vi "_Pull Controls Value to DPs(VI).vi"(6 "sync DPs?(T)":bool=TRUE, 7 "VIRef(Caller VI)":refnum<vi>, 8 "error in (no error)":errorcluster, 9 "force update(F)":bool, 11 "SILAPI In":refnum<k1>) -> (0 "error out":errorcluster, 1 "Binded DPs":string[](array[string]), 3 "SILAPI Out":refnum<k1>)   [LabVIEW 2017, in "TagDB RefManager.lvlib"]
uses:
  TagDB RefManager.lvlib
  230c0da9-b6e4-44e0-8cb2-fe6bdec026ba.vi
  e135edd7-4a87-4b9d-b0c7-3b3f0cd11366.vi
  be640558-f0fc-44bb-96cd-108508b5fbdb.vi
  083faeab-0307-4387-9797-c882d96e285b.vi
  a032c900-6a26-4ad4-8296-bdd15205f1fc.vi
  024ec822-42c1-4cee-abf5-dbe2fbe4f70a.vi
  <userlib>/_NEVSTOP/TagDB/_Support/DataAccess/_NameCacher.vi
  <userlib>/_NEVSTOP/TagDB/_Support/Error/_[error50002]Invalid DataType.vi
  <userlib>/_NEVSTOP/TagDB/_Support/Error/_[error50000]Invalid DB REF.vi
  <userlib>/_NEVSTOP/TagDB/_Support/DataAccess/TagDB Ref to DVR.vi
  <userlib>/_NEVSTOP/TagDB/_Support/URL/TRIM-BOTH-SPACE.vi
  <userlib>/_NEVSTOP/TagDB/_Support/DataAccess/data-Write.vi
  <userlib>/_NEVSTOP/TagDB/_Support/DataAccess/_datatypeChecker.vi
  <userlib>/_NEVSTOP/TagDB/_Support/Error/_Build Error Cluster.vi
  <vilib>/Utility/Data Type/Get Type Information.vi
  <userlib>/_NEVSTOP/TagDB/TagDB.lvlib
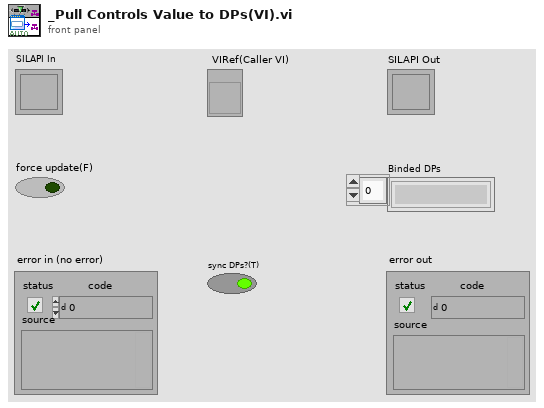
[diagram p1: front panel]
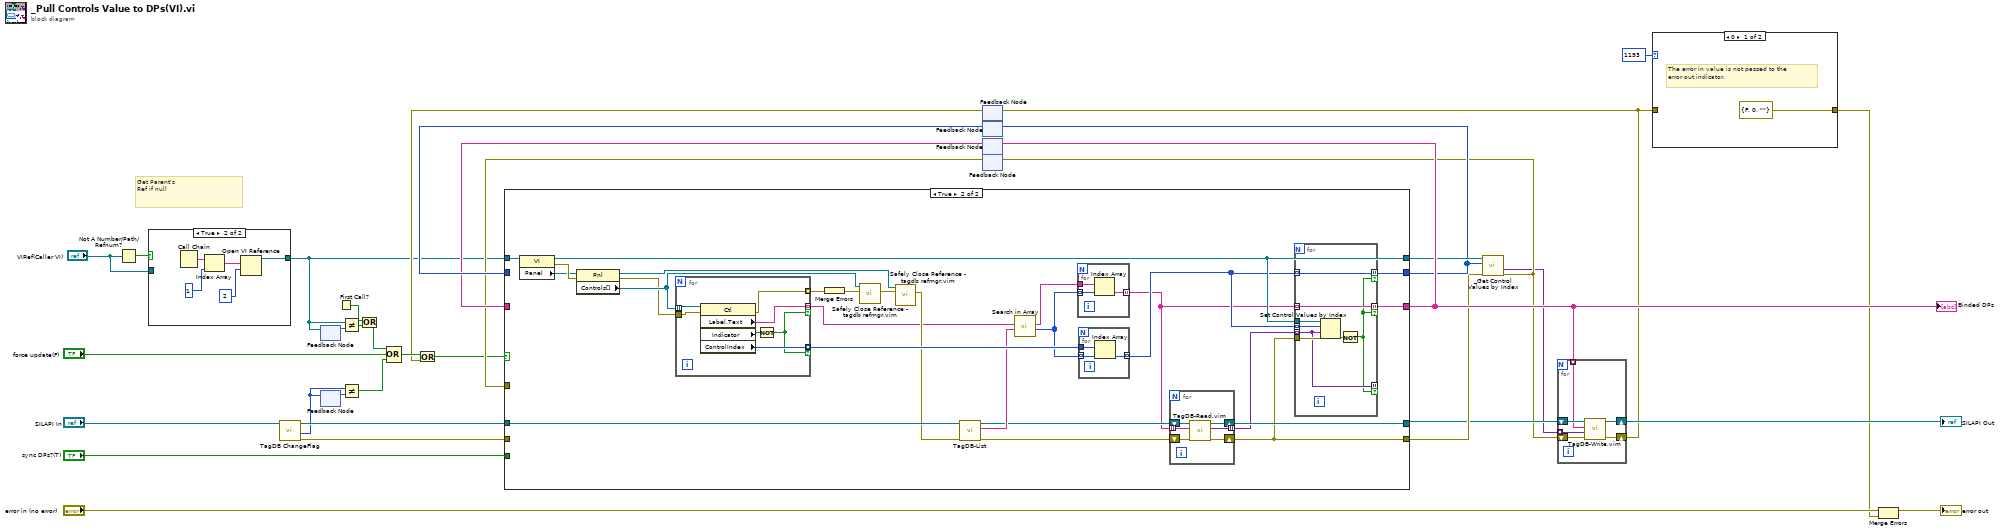
[diagram p0: block diagram]
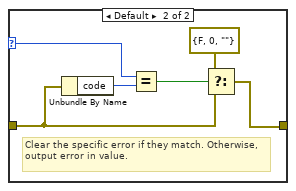
[diagram p3: hidden frame]
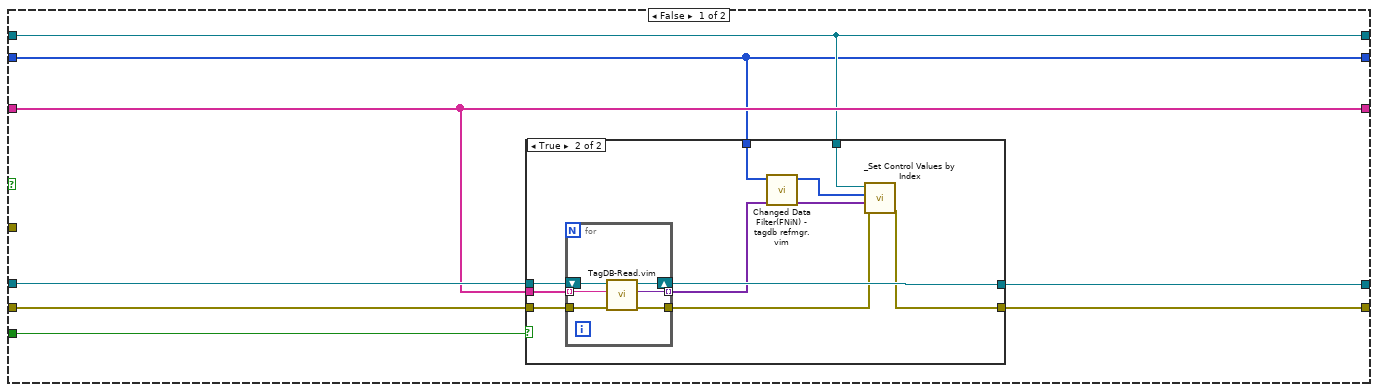
[diagram p4: hidden frame]
diagram:
  # "Get Parent's\nRef if null"
  n1 = Not A Number/Path/Refnum?(number/path/refnum="VIRef(Caller VI)") -> (NaN/Path/Refnum?=w13:bool)
  n2 = case shown="True" w13 {
    tunnel: [w35 w36] -> w8
    tunnel: "VIRef(Caller VI)" -> [w35 _]
    frame False {
    }
    frame True {
      n3 = Call Chain() -> (call chain=w40:string[])
      n4 = Index Array(array=w40, index=1 ("Index")) -> (element=w38:string)
      n5 = Open VI Reference(vi path=w38, options=2) -> (vi reference=w36:refnum<vi>)  [unwired: 4 in, 1 out]
    }
  }
  n6 = call <userlib>:"TagDB ChangeFlag.vi"("DB Ref"="SILAPI In") -> ("error in (no error) (dup)"=w3:errorcluster, "Item Change Timestamp"=w5:u64, "DB Ref (dup)"=w7:refnum<k1>)  [unwired: 7 in, 1 out]
  n7 = feedback #1() -> (w12:refnum<vi>)  [unwired: 1 in]
  n8 = feedback-in #1(w8) -> ()
  n9 = feedback #2() -> (w6:u64)  [unwired: 1 in]
  n10 = feedback-in #2(w5) -> ()
  n11 = First Call?() -> (First Call?: T/F=w10:bool)
  n12 = Not Equal?(x=w8, y=w12) -> (x != y?=w11:bool)
  n13 = Not Equal?(x=w5, y=w6) -> (x != y?=w4:bool)
  n14 = Or(x=w10, y=w11) -> (x .or. y?=w9:bool)
  n15 = Compound Arithmetic op=OR(w9, "force update(F)", w4) -> (w23:bool)
  n16 = feedback #3() -> (w18:errorcluster)  [unwired: 1 in]
  n17 = Or(x=w23, y=w18) -> (x .or. y?=w19:bool)
  n18 = feedback #4() -> (w24:i32[])  [unwired: 1 in]
  n19 = feedback #5() -> (w22:string[])  [unwired: 1 in]
  n20 = feedback #6() -> (w21:errorcluster)  [unwired: 1 in]
  n21 = case shown="True" w19 {
    tunnel: [w45 w83] -> w26
    tunnel: w8 -> [w45 w93]
    tunnel: [w43 w86] -> w25
    tunnel: w24 -> [w43 _]
    tunnel: [w47 w87] -> w29
    tunnel: w22 -> [w47 _]
    tunnel: w7 -> [w48 w92]
    tunnel: [w44 w88] -> w16
    tunnel: w21 -> [_ _]
    tunnel: [w46 w90] -> w15
    tunnel: "sync DPs?(T)" -> [w42 _]
    tunnel: w3 -> [w41 _]
    frame False {
      n22 = case shown="True" w42 {
        tunnel: w48 -> [w50 w61]
        tunnel: w47 -> [_ w60]
        tunnel: [w50 w59] -> w46
        tunnel: w45 -> [_ w58]
        tunnel: [w49 w56] -> w44
        tunnel: w43 -> [_ w53]
        tunnel: w41 -> [w49 w51]
        frame False {
        }
        frame True {
          n23 = for {
            tunnel: w60 -> [w66] mode=indexing
            tunnel: [w64] -> w57
            tunnel: [w63] -> w55 mode=indexing
            shift-right: [w65] -> w59
            shift-left: w61 -> [w67]
            tunnel: w51 -> [w62]
            n24 = call "TagDB-Read.vim"("error in (no error)"=w62, "name"=w66, "TagDB"=w67) -> ("error out"=w64:errorcluster, "Value"=w63:variant, "TagDB(dup)"=w65:refnum<k1>)  [unwired: 3 in, 3 out]
          }
          n25 = call "Changed Data Filter(FNiN) - tagdb refmgr.vim"("checked data"=w55, "1"=w53) -> ("data"=w54:variant[], "1 out"=w52:i32[])  [unwired: 6 in, 2 out]
          n26 = call <userlib>:"_Set Control Values by Index.vi"("error in (no error)"=w57, "data values"=w54, "control indexes"=w52, "VI Refnum"=w58) -> ("error out"=w56:errorcluster)  [unwired: 7 in]
        }
      }
    }
    frame True {
      n27 = property class="VI"(reference=w93) -> (reference out=w83:refnum<vi>, error out=w85:errorcluster, "Panel"=w84:refnum<vi>)  [unwired: 1 in]
      n28 = property class="Pnl"(reference=w84, error in=w85) -> (reference out=w77:refnum<vi>, error out=w74:errorcluster, "Controls[]"=w79:refnum<vi>[])
      n29 = for {
        tunnel: w79 -> [w112] mode=indexing
        tunnel: [w111] -> w71 mode=indexing if=w106
        tunnel: [w110] -> w82 mode=indexing if=w106
        tunnel: [w108] -> w80 mode=indexing
        tunnel: w74 -> [w107]
        n30 = property class="Ctl"(reference=w112, error in=w107) -> (error out=w108:errorcluster, "Label.Text"=w111:string, "Indicator"=w109:bool, "ControlIndex"=w110:i32)  [unwired: 1 out]
        n31 = Not(x=w109) -> (.not. x?=w106:bool)
      }
      n32 = Merge Errors(w80) -> (w78:errorcluster)
      n33 = call "Safely Close Reference - tagdb refmgr.vim"("error in (no error)"=w78, "Reference"=w79) -> ("error out"=w76:errorcluster)  [unwired: 9 in]
      n34 = call "Safely Close Reference - tagdb refmgr.vim"("error in (no error)"=w76, "Reference"=w77) -> ("error out"=w75:errorcluster)  [unwired: 9 in]
      n35 = call <userlib>:"TagDB-List.vi"("error in (no error)"=w75, "TagDB"=w92) -> ("error out"=w91:errorcluster, "names"=w73:string[], "TagDB(dup)"=w72:refnum<k1>)  [unwired: 6 in, 1 out]
      n36 = call "Search in Array.vi"("items to filter"=w73, "array"=w71) -> ("item Indexs"=w70:i32[], "array(dup)"=w68:string[])  [unwired: 4 in]
      n37 = for {
        tunnel: w70 -> [w96] mode=indexing
        tunnel: w68 -> [w95]
        tunnel: [w94] -> w69 mode=indexing
        n38 = Index Array(array=w95, index=w96) -> (element=w94:string)
      }
      n39 = for {
        tunnel: w70 -> [w99] mode=indexing
        tunnel: w82 -> [w98]
        tunnel: [w97] -> w81 mode=indexing
        n40 = Index Array(array=w98, index=w99) -> (element=w97:i32)
      }
      n41 = for {
        tunnel: [w103] -> w89 mode=indexing
        tunnel: w69 -> [w101] mode=indexing
        shift-right: [w102] -> w88
        shift-left: w91 -> [w105]
        shift-right: [w104] -> w90
        shift-left: w72 -> [w100]
        n42 = call "TagDB-Read.vim"("error in (no error)"=w105, "name"=w101, "TagDB"=w100) -> ("error out"=w102:errorcluster, "Value"=w103:variant, "TagDB(dup)"=w104:refnum<k1>)  [unwired: 3 in, 3 out]
      }
      n43 = for {
        tunnel: w83 -> [w120]
        tunnel: w81 -> [w119] mode=indexing
        tunnel: w89 -> [w115] mode=indexing
        tunnel: w88 -> [w118]
        tunnel: [w117] -> w87 mode=indexing if=w113
        tunnel: w69 -> [w117] mode=indexing
        tunnel: [w116] -> w86 mode=indexing if=w113
        tunnel: w81 -> [w116] mode=indexing
        tunnel: [w115] -> _ mode=indexing if=w113
        n44 = Set Control Values by Index(0:w120, 1:w119, 2:w115, 3:w118) -> (11:w114:errorcluster)
        n45 = Not(x=w114) -> (.not. x?=w113:bool)
      }
    }
  }
  "Binded DPs" <- w29
  n46 = feedback-in #4(w25) -> ()
  n47 = feedback-in #5(w29) -> ()
  n48 = call <userlib>:"_Get Control Values by Index.vi"("error in (no error)"=w16, "control indexes"=w25, "VI Refnum"=w26) -> ("error out"=w2:errorcluster, "data values"=w1:variant[])  [unwired: 7 in]
  n49 = feedback-in #6(w2) -> ()
  n50 = for {
    tunnel: w1 -> [w122] mode=indexing
    shift-right: [w125] -> w30
    shift-left: w15 -> [w126]
    shift-right: [w123] -> w14
    shift-left: w2 -> [w124]
    tunnel: w29 -> [w121] mode=indexing
    n51 = call "TagDB-Write.vim"("error in (no error)"=w124, "Value"=w122, "tag"=w121, "TagDB"=w126) -> ("error out"=w123:errorcluster, "TagDB(dup)"=w125:refnum<k1>)  [unwired: 5 in, 1 out]
  }
  "SILAPI Out" <- w30
  n52 = feedback-in #3(w14) -> ()
  n53 = case shown="0" 1193 ("specific error code to clear (0: all)") {
    selector: 1193 ("specific error code to clear (0: all)") -> [_ w132]
    tunnel: w14 -> [_ w131]
    tunnel: [errorcluster {"status"=FALSE, "code"=0, "source"=""} ("error constant") w128] -> w20
    frame 0 {
      # "The error in value is not passed to the\nerror out indicator."
    }
    frame Default {
      # "Clear the specific error if they match. Otherwise, output error in value."
      n54 = Unbundle By Name(w131) -> ("code"=w133:i32)
      n55 = Equal?(x=w132, y=w133) -> (x = y?=w129:bool)
      n56 = Select(t=errorcluster {"status"=FALSE, "code"=0, "source"=""} ("error constant"), s=w129, f=w131) -> (s? t:f=w128:errorcluster)
    }
  }
  n57 = Merge Errors("error in (no error)", w20) -> (→"error out":errorcluster)
